vi "CE - PSD Trace Type.vi"(8 "error in (no error)":errorcluster, 11 "SA Measurement in":refnum<class "SA Measurement.lvclass">) -> (0 "error out":errorcluster, 3 "SA Measurement out":refnum<class "SA Measurement.lvclass">)   [LabVIEW 2023, in "Spectrum Analyzer.lvlib" / "SA Measurement.lvclass"]
uses:
  SA Measurement.lvclass
  Keysight 9020A/Keysight 9020A.lvclass
  D:/Project/IST013_CE Conduction Measurement/IST013-CE-Condcuted-Measurement/src/Spectrum Analyzer/Interface_Spectrum/Interface_Spectrum.lvclass
  TYPE DEFINITION/SA Measurement Class/TYPE CE PSD Setting Parameter.ctl
  TYPE DEFINITION/TYPE Y-axis Unit.ctl
  TYPE DEFINITION/TYPE Start and Stop Frequency.ctl
  TYPE DEFINITION/TYPE Center and Span Frequency.ctl
  TYPE DEFINITION/TYPE Reference Level and Atten Param.ctl
  TYPE DEFINITION/TYPE Display Trace Mode Select.ctl
  TYPE DEFINITION/TYPE Detect Mode Select.ctl
  TYPE DEFINITION/TYPE Average Mode Select.ctl
  Keysight 9020A/Keysight 9020A.lvclass/Keysight 9020A.ctl
  SA Measurement.lvclass/SA Measurement.ctl
  Spectrum Analyzer.lvlib
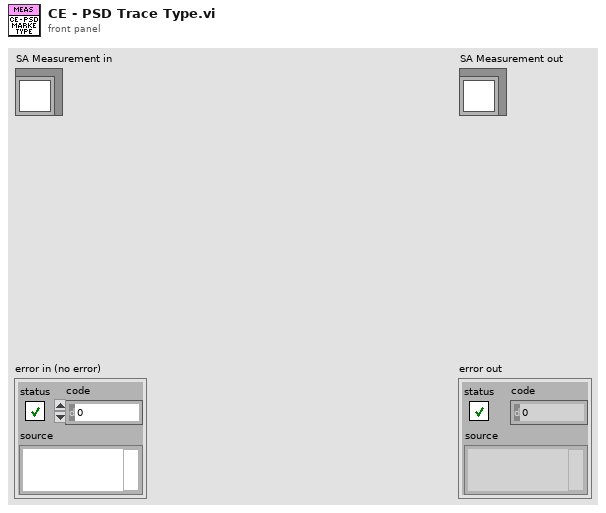
[diagram p1: front panel]
types:
  T1 = typedef "Spectrum Analyzer.lvlib/TYPE CE PSD Setting Parameter.ctl" = cluster{"Y-axis Unit":T2, "Start/Stop Frequency(Hz)":T3, "Center and Span Frequency(Hz)":T4, "PSD Type":enum16{"Marker", "Trace"}, "Ref and Atten":T5, "External Loss":dbl, "RBW/VBW(Hz)":cluster{"RBW":dbl, "VBW":dbl}, "Sweep Point":u32, "Sweep Time(s)":cluster{"Time":dbl, "Auto?":bool}, "Trace and Detect":cluster{"Trace Mode":T6, "Detector Type":T7, "Detect Auto?":bool}[], "Average Mode":T8, "Avg/Hold Number":u32}
  T2 = typedef "Spectrum Analyzer.lvlib/TYPE Y-axis Unit.ctl" = enum16{"dBm", "dBmV", "dBuV", "dBpW", "Volt", "Ampere", "Watt"}
  T3 = typedef "Spectrum Analyzer.lvlib/TYPE Start and Stop Frequency.ctl" = cluster{"Start":dbl, "Stop":dbl}
  T4 = typedef "Spectrum Analyzer.lvlib/TYPE Center and Span Frequency.ctl" = cluster{"Center":dbl, "Span":dbl}
  T5 = typedef "Spectrum Analyzer.lvlib/TYPE Reference Level and Atten Param.ctl" = cluster{"Reference Level":dbl, "Atten":i32, "Atten Auto?":bool}
  T6 = typedef "Spectrum Analyzer.lvlib/TYPE Display Trace Mode Select.ctl" = enum16{"Clear Write", "Max Hold", "Min Hold", "Average", "View"}
  T7 = typedef "Spectrum Analyzer.lvlib/TYPE Detect Mode Select.ctl" = enum16{"Det Auto (Normal)", "Auto Peak", "Positive Peak", "Negative Peak", "Sample", "RMS", "Average", "Quasipeak", "CISPR Average", "RMS Average"}
  T8 = typedef "Spectrum Analyzer.lvlib/TYPE Average Mode Select.ctl" = enum16{"Linear(Voltage Avg)", "Video(Log)", "Power"}
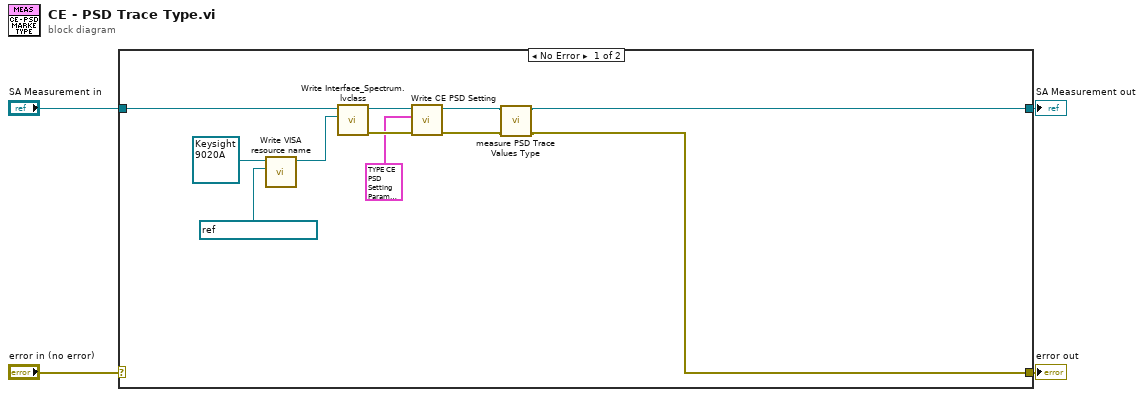
[diagram p0: block diagram]
diagram:
  n1 = case shown="No Error" "error in (no error)" {
    selector: "error in (no error)" -> [_ w17]
    tunnel: [w5 w17] -> w3
    tunnel: [w6 w16] -> w1
    tunnel: "SA Measurement in" -> [w13 w16]
    frame No Error {
      n2 = call "Write VISA resource name.vi"("VISA resource name"=refnum<visa-resource-name> "GPIB0::18::INSTR", "Keysight 9020A in"=refnum<class "Keysight 9020A.lvclass"> refnum ("Spectrum Analyzer.lvlib:Keysight 9020A.lvclass")) -> ("Keysight 9020A out"=w12:refnum<class "Keysight 9020A.lvclass">)  [unwired: 8 in, 1 out]
      n3 = call "Write Interface_Spectrum.lvclass.vi"("Interface_Spectrum.lvclass"=w12, "SA Measurement in"=w13) -> ("error out"=w10:errorcluster, "SA Measurement out"=w11:refnum<class "SA Measurement.lvclass">)  [unwired: 8 in]
      n4 = call "Write CE PSD Setting.vi"("error in (no error)"=w10, "CE PSD Setting"=T1 {"Y-axis Unit"=enum."dBm", "Start/Stop Frequency(Hz)"={"Start"=2400000000.0, "Stop"=2483500000.0}, "Center and Span Frequency(Hz)"={"Center"=2412000000.0, "Span"=20000000.0}, "PSD Type"=enum."Trace", "Ref and Atten"={"Reference Level"=0.0, "Atten"=20, "Atten Auto?"=FALSE}, "External Loss"=10.0, "RBW/VBW(Hz)"={"RBW"=10000.0, "VBW"=3000.0}, "Sweep Point"=8351, "Sweep Time(s)"={"Time"=10.0, "Auto?"=FALSE}, "Trace and Detect"=[{"Trace Mode"=enum."Max Hold", "Detector Type"=enum."Average", "Detect Auto?"=FALSE}], "Average Mode"=enum."Power", "Avg/Hold Number"=2}, "SA Measurement in"=w11) -> ("error out"=w7:errorcluster, "SA Measurement out"=w8:refnum<class "SA Measurement.lvclass">)  [unwired: 7 in]
      n5 = call "measure PSD Trace Values Type.vi"("error in (no error)"=w7, "SA Measurement in"=w8) -> ("error out"=w5:errorcluster, "SA Measurement out"=w6:refnum<class "SA Measurement.lvclass">)  [unwired: 8 in]
    }
    frame Error {
    }
  }
  "error out" <- w3
  "SA Measurement out" <- w1
